vi "Own20261012_SetControlIndicator.vi"() -> ()   [LabVIEW 2024]
panel:
  out "error out":errorcluster caption="错误输出"
  in  "is_indicator":bool
  in  "control_id":u32
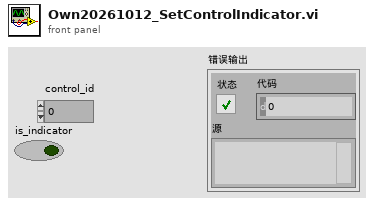
[diagram p1: front panel]
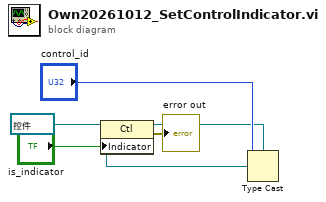
[diagram p0: block diagram]
diagram:
  n1 = Type Cast(type=refnum<vi> refnum ("引用"), x="control_id") -> (*(type *) &x=w3:refnum<vi>)
  n2 = property class="Ctl"(reference=w3, "Indicator"="is_indicator") -> (error out=→"error out":errorcluster)  [unwired: 1 in, 1 out]
